vi "GetMCLBHeaders.vi"(0 "Ctl Refnum In":refnum<vi>, 11 "Error In":errorcluster) -> (4 "Ctl Refnum Out":refnum<vi>, 6 "Row Headers":string[](array[string]), 8 "Column Headers":string[](array[string]), 15 "Error Out":errorcluster)   [LabVIEW 2019, in "Drona.lvlib"]
doc: "This VI gives MCLB rows and column headers"
uses:
  Drona.lvlib
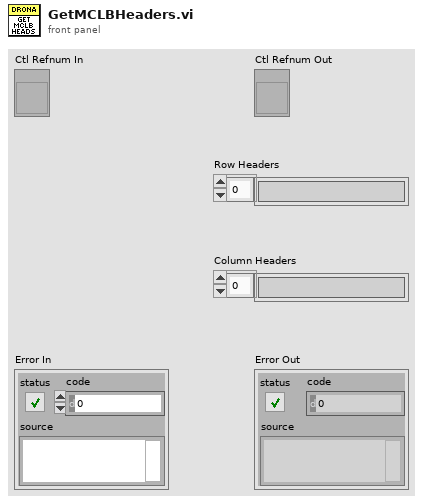
[diagram p1: front panel]
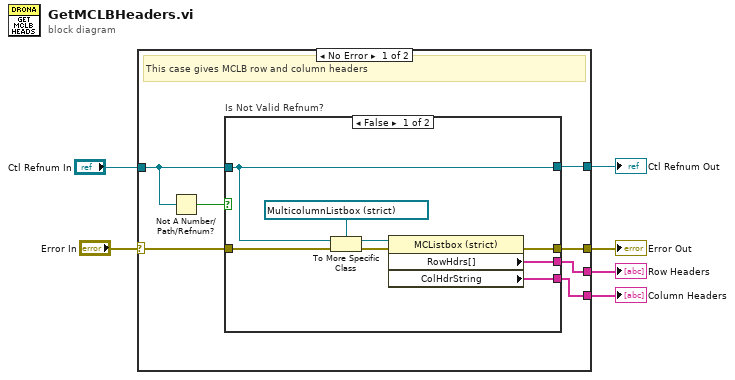
[diagram p0: block diagram]
diagram:
  n1 = case shown="No Error" "Error In" {
    selector: "Error In" -> [w13 w24]
    tunnel: "Ctl Refnum In" -> [w10 w25]
    tunnel: [w9 w25] -> w4
    tunnel: [w11 w24] -> w3
    tunnel: [w8 _] -> w2
    tunnel: [w7 _] -> w1
    frame No Error {
      # "This case gives MCLB row and column headers"
      n2 = Not A Number/Path/Refnum?(number/path/refnum=w10) -> (NaN/Path/Refnum?=w12:bool)
      n3 = case "Is Not Valid Refnum?" shown="False" w12 {
        tunnel: w13 -> [w21 w23]
        tunnel: [w18 w23] -> w11
        tunnel: w10 -> [w19 w22]
        tunnel: [w19 w22] -> w9
        tunnel: [w16 _] -> w8
        tunnel: [w15 _] -> w7
        frame False {
          n4 = To More Specific Class(target class=refnum<vi> refnum ("Multicolumn Listbox"), reference=w19, error in=w21) -> (specific class reference=w17:refnum<vi>, error out=w20:errorcluster)
          n5 = property class="MCListbox (strict)"(reference=w17, error in=w20) -> (error out=w18:errorcluster, "RowHdrs[]"=w16:string[], "ColHdrString"=w15:string[])  [unwired: 1 out]
        }
        frame True {
        }
      }
    }
    frame Error {
      # "If error, this case pass that error messge only"
    }
  }
  "Ctl Refnum Out" <- w4
  "Error Out" <- w3
  "Row Headers" <- w2
  "Column Headers" <- w1
